vi "Control_1_15.vi"() -> ()   [LabVIEW 2025]
uses:
  <vilib>/addons/zeromq/socket_type.ctl
  <vilib>/DAQmx/write.llb/DAQmx Write (Analog 1D DBL NChan 1Samp).vi
  <vilib>/DAQmx/read.llb/DAQmx Read (Analog DBL 1Chan 1Samp).vi
  <vilib>/DAQmx/read.llb/DAQmx Read (Analog 1D DBL NChan 1Samp).vi
  <vilib>/DAQmx/create/channels.llb/DAQmx Create Channel (AI-Voltage-Basic).vi
  Trimming_Coil_Monitor.vi
  <vilib>/Waveform/DWDTOps.llb/DWDT Digital to Boolean Array.vi
  Trimming_Coil_Command.vi
  <vilib>/DAQmx/miscellaneous.llb/DAQmx Fill In Error Info.vi
  <vilib>/DAQmx/create/channels.llb/DAQmx Create Channel (AO-Voltage-Basic).vi
  Trimming_Coil_Ramps.vi
  <vilib>/addons/zeromq/zmq_socket.lvclass
  <vilib>/addons/zeromq/zmq_context.lvclass
  <vilib>/addons/zeromq/zeromq.lvlib
  <resource>/objmgr/daqmx.rc
panel:
  out "TC6_Ramp":dbl
  out "TC7_Ramp":dbl
  out "x*y":dbl[](array[numeric])
  in  "stop":bool
  out "TC9_Ramp":dbl
  out "TC6_Set_Point":dbl
  out "TC5_Ramp":dbl
  out "TC10_Ramp":dbl
  in  "RF":tag
  in  "Others":tag
  out "error out":errorcluster
  out "double precision float":dbl
  out "Source 1":dbl
  out "Source 2":dbl
  out "Source 3":dbl
  out "Source 4":dbl
  out "Source 5":dbl
  out "Source 6":dbl
  out "Source 7":dbl
  out "Source 8":dbl
  out "Source 9":dbl
  out "Source 10":dbl
  out "Source 11":dbl
  out "Source 12":dbl
  out "Source 13":dbl
  out "Source 14":dbl
  out "value":dbl[](array[numeric])
  out "subarray":dbl[](array[numeric])
  out "Boolean array":bool[](array[boolean])
  out "TC 7":dbl
  out "TC 8":dbl
  in  "Boolean":bool
  out "Array":dbl[](array[numeric])
  out "max value":i16
  out "Array[0]":dbl
  out "Array 2":dbl[](array[numeric])
  in  "TP1":dbl
  in  "TP2":dbl
  in  "RF 2":dbl
  in  "Beam":dbl
  in  "Boolean 2":bool
  in  "Boolean 3":bool
  out "[0]":bool
  out "[1]":bool
  out "[2]":bool
  out "[3]":bool
  out "others":dbl[](array[numeric]) format="%0.2f"
  out "TC1_SP":dbl
  # "Beam I"
  # "ESD KV"
  # "ARC V"
  # "Filament C"
  # "Inside Iron"
  # "Outside Iron"
  # "ARC C"
  # "ESD mA"
  # "TC1"
  # "TC2"
  # "TC4"
  # "TC5"
  # "TC6"
  # "TC7"
  # "TC10"
  # "TC9"
  # "TP2"
  # "TP1"
  # "Filament V"
  # "Centering Beam"
  # "TC 12"
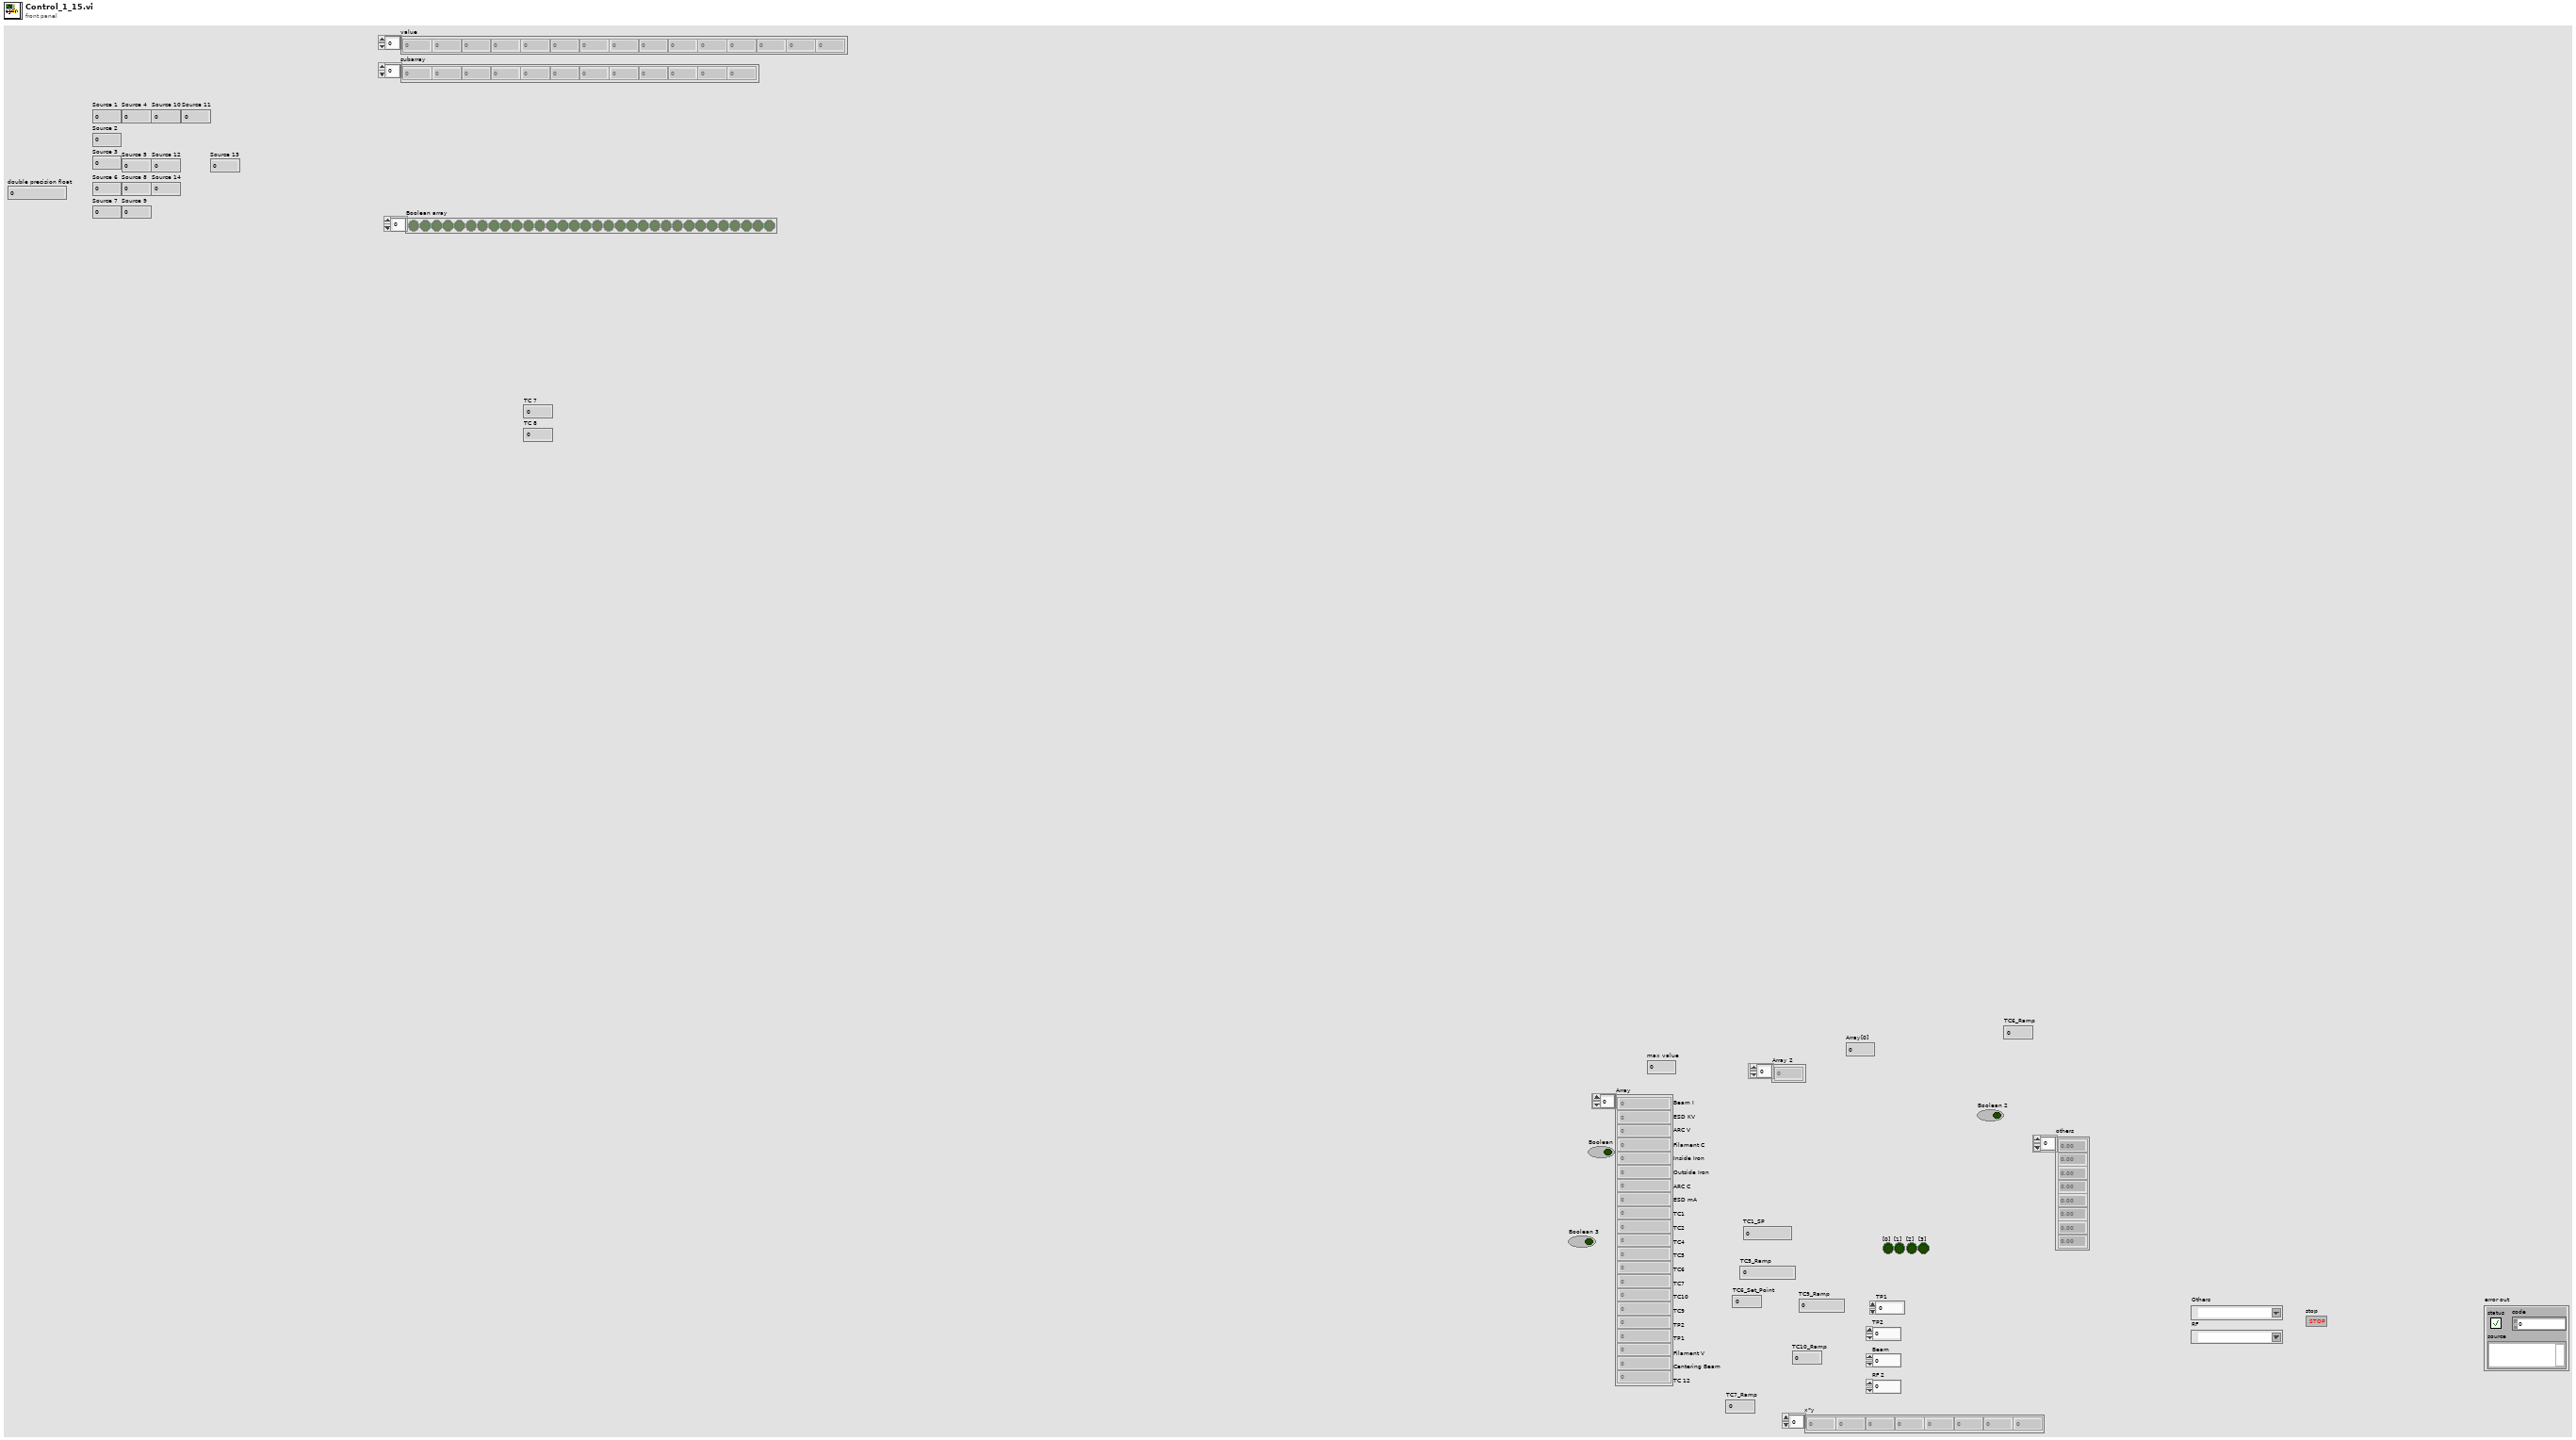
[diagram p1: front panel]
types:
  T1 = typedef "zeromq.lvlib/socket_type.ctl" = enum8{"ZMQ_PAIR", "ZMQ_PUB", "ZMQ_SUB", "ZMQ_REQ", "ZMQ_REP", "ZMQ_DEALER", "ZMQ_ROUTER", "ZMQ_PULL", "ZMQ_PUSH", "ZMQ_XPUB", "ZMQ_XSUB", "ZMQ_STREAM", "ZMQ_SERVER", "ZMQ_CLIENT", "ZMQ_RADIO", "ZMQ_DISH", "ZMQ_GATHER", "ZMQ_SCATTER", "ZMQ_DGRAM"}
  T2 = enum16{"big-endian, network order", "native, host order", "little-endian"}
  T3 = cluster{"[0]":dbl, "[1]":dbl, "[2]":dbl, "[3]":dbl, "[4]":dbl, "[5]":dbl, "[6]":dbl, "[7]":dbl}
  T4 = cluster{"Array[0]":dbl, "Array[1]":dbl, "Array[2]":dbl, "Array[3]":dbl, "Array[4]":dbl, "Array[5]":dbl, "Array[6]":dbl, "Array[7]":dbl}
  T5 = cluster{"[0]":digitalwaveform, "[1]":digitalwaveform, "[2]":digitalwaveform, "[3]":digitalwaveform, "[4]":digitalwaveform, "[5]":digitalwaveform, "[6]":digitalwaveform, "[7]":digitalwaveform, "[8]":digitalwaveform}
  T6 = cluster{"TC1_Readback":dbl, "TC2_Readback":dbl, "TC3_Readback":dbl, "TC4_Readback":dbl, "TC5_Readback":dbl, "TC6_Readback":dbl, "TC7_Readback":dbl, "TC8_Readback":dbl, "TC9_Readback":dbl, "TC10_Readback":dbl, "TC11_Readback":dbl, "TC12_Readback":dbl}
  T7 = cluster{"[0]":bool, "[1]":bool, "[2]":bool, "[3]":bool, "[4]":bool, "[5]":bool, "[6]":bool, "[7]":bool, "[8]":bool}
  T8 = cluster{"TC1_Set_Point":dbl, "TC2_Set_Point":dbl, "TC3_Set_Point":dbl, "TC4_Set_Point":dbl, "TC5_Set_Point":dbl, "TC6_Set_Point":dbl, "TC7_Set_Point":dbl, "TC8_Set_Point":dbl, "TC9_Set_Point":dbl, "TC10_Set_Point":dbl, "TC11_Set_Point":dbl, "TC12_Set_Point":dbl}
  T9 = cluster{"TC1_Ramp":dbl, "TC2_Ramp":dbl, "TC3_Ramp":dbl, "TC4_Ramp":dbl, "TC5_Ramp":dbl, "TC6_Ramp":dbl, "TC7_Ramp":dbl, "TC8_Ramp":dbl, "TC9_Ramp":dbl, "TC10_Ramp":dbl, "TC11_Ramp":dbl, "TC12_Ramp":dbl}
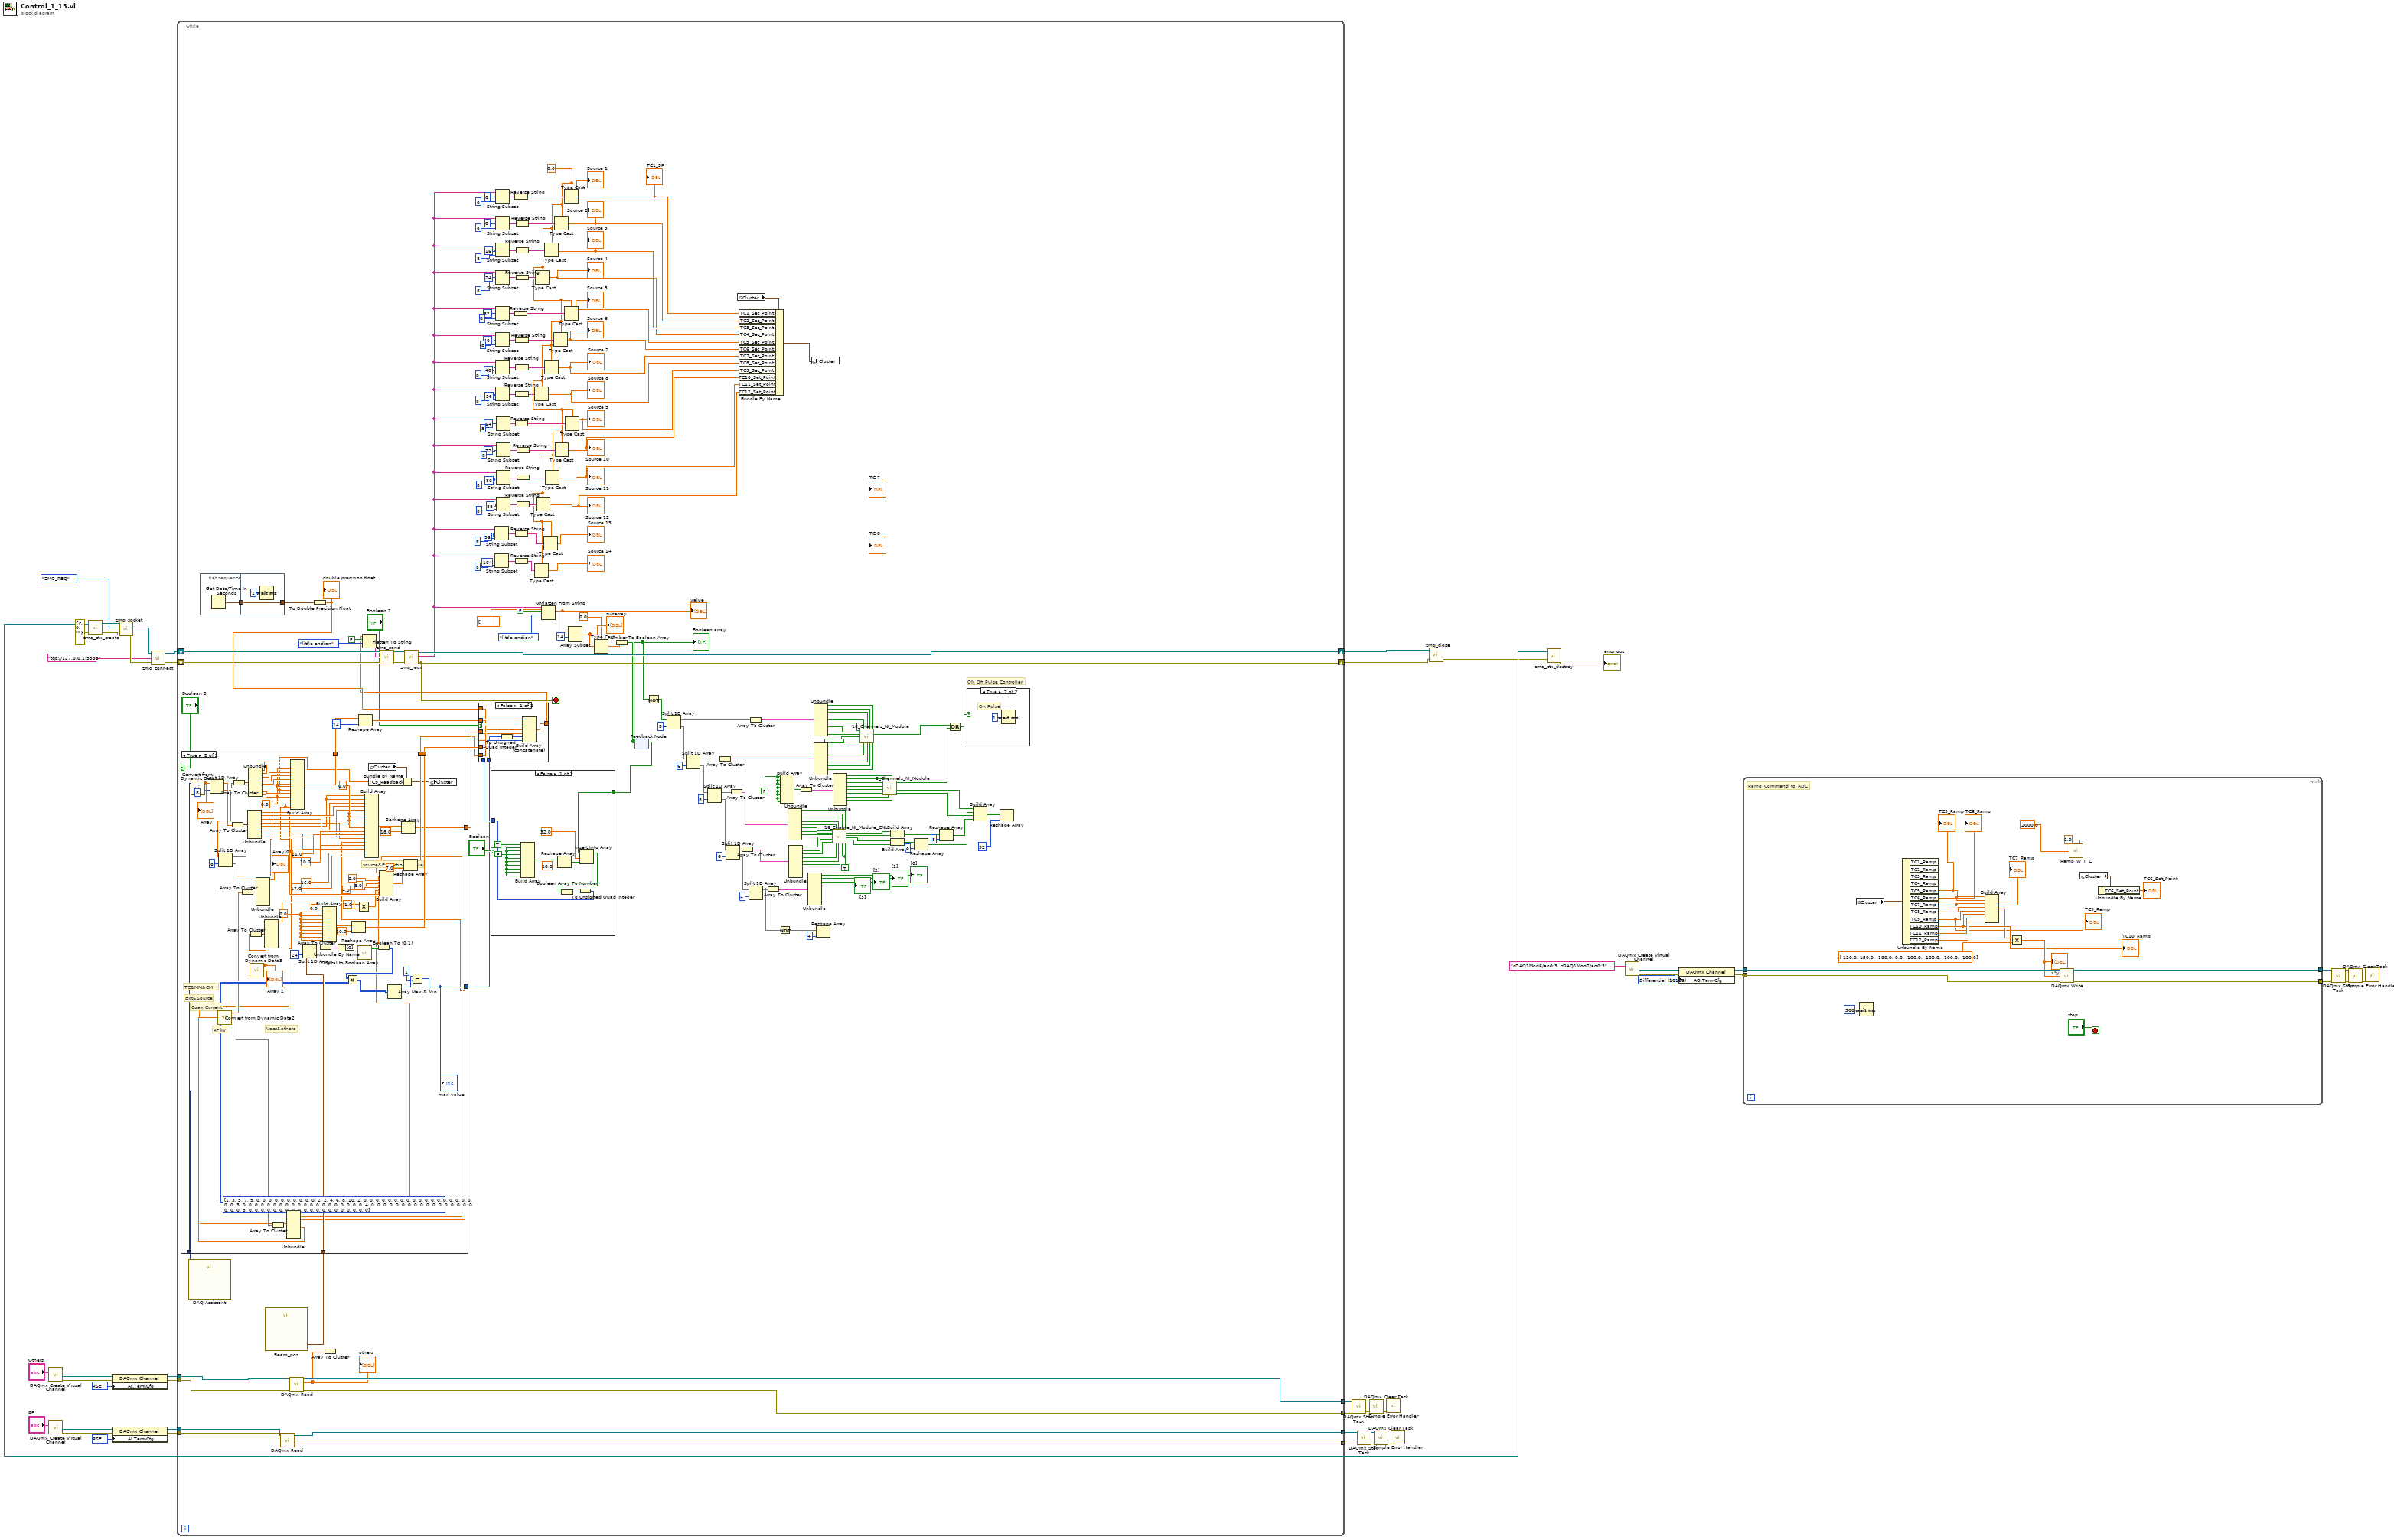
[diagram p0: block diagram]
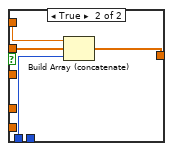
[diagram p2: hidden frame]
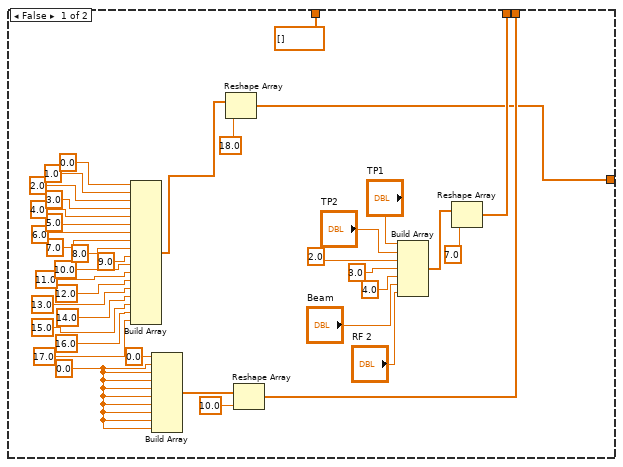
[diagram p3: hidden frame]
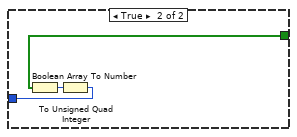
[diagram p4: hidden frame]
diagram:
  w8 = 10106 items=["RSE"=10083, "Differential"=10106, "Pseudodifferential"=12529] ("AO.TermCfg")
  w20 = 10083 items=["RSE"=10083, "Differential"=10106, "Pseudodifferential"=12529] ("AO.TermCfg")
  w31 = 10083 items=["RSE"=10083, "Differential"=10106, "Pseudodifferential"=12529] ("AO.TermCfg")
  n1 = call-poly <vilib>:"DAQmx Create Virtual Channel.vi"("physical channels"="Others") -> ("task out"=w32:refnum<k21>, "error out"=w33:errorcluster)  [unwired: 13 in]
  n2 = call-poly <vilib>:"DAQmx Create Virtual Channel.vi"("physical channels"="RF") -> ("task out"=w21:refnum<k21>, "error out"=w22:errorcluster)  [unwired: 13 in]
  n3 = call <vilib>:"zmq_ctx_create.vi"("error in"=errorcluster {"status"=FALSE, "code"=0, "source"=""}) -> ("error out"=w45:errorcluster, "context out"=w46:refnum<class "zmq_context.lvclass">)  [unwired: 3 in]
  n4 = property class="DAQmx Channel"(reference=w32, error in=w33, "AI.TermCfg"=w31) -> (reference out=w26:refnum<k21>, error out=w25:errorcluster)
  n5 = property class="DAQmx Channel"(reference=w21, error in=w22, "AI.TermCfg"=w20) -> (reference out=w18:refnum<k21>, error out=w17:errorcluster)
  n6 = call <vilib>:"zmq_socket.vi"("error in"=w45, "socket type"=socket_type."ZMQ_REQ", "context in"=w46) -> ("error out"=w43:errorcluster, "socket out"=w44:refnum<class "zmq_socket.lvclass">, "context out"=w38:refnum<class "zmq_context.lvclass">)  [unwired: 2 in]
  n7 = call <vilib>:"zmq_connect.vi"("error in"=w43, "endpoint"="tcp://127.0.0.1:5555", "socket in"=w44) -> ("error out"=w39:errorcluster, "socket out"=w40:refnum<class "zmq_socket.lvclass">)  [unwired: 1 in]
  n8 = while {
    shift-right: [w177] -> w35
    shift-left: w40 -> [w251]
    shift-right: [w176] -> w36
    shift-left: w39 -> [w250]
    tunnel: w26 -> [w77]
    tunnel: w25 -> [w76]
    tunnel: [w75] -> w24
    tunnel: [w74] -> w23
    tunnel: w18 -> [w73]
    tunnel: w17 -> [w72]
    tunnel: [w71] -> w13
    tunnel: [w70] -> w12
    stop <- w176 stop-if-true
    w104 = TRUE
    w107 = FALSE
    w62 = 0.0
    # "ON_Off Pulse Controller"
    n9 = call "DAQ Assistant"() -> ("data"=w64:dynamicdata)  [unwired: 16 in, 3 out]
    n10 = flat-sequence {
      tunnel: [w391] -> w246
      tunnel: [w393] -> w247
      tunnel: w246 -> [w393]
      frame #0 {
        n11 = Get Date/Time In Seconds() -> (seconds since 1Jan1904=w391:timestamp)
      }
      frame #1 {
        n12 = Wait (ms)(milliseconds to wait=u32 1) -> ()  [unwired: 1 out]
      }
    }
    n13 = call "Beam_pos"() -> ("data"=w65:digitalwaveform[])  [unwired: 16 in, 3 out]
    n14 = case shown="True" "Boolean 3" {
      tunnel: [w276 w365] -> w92
      tunnel: [w270 w360] -> w91
      tunnel: [w273 w363] -> w90
      tunnel: w64 -> [_ w357]
      tunnel: [dbl[] [] w358] -> w67
      tunnel: w65 -> [_ w340]
      tunnel: [_ w328] -> w63
      frame False {
        w277 = 0.0 ("element")
        n15 = Build Array(0.0, 1.0, 2.0, 3.0, 4.0, 5.0, 6.0, 7.0, 8.0, 9.0, 10.0, 11.0, 12.0, 13.0, 14.0, 15.0, 16.0, 17.0) -> (w271:dbl[])
        n16 = Build Array(0.0 ("element"), w277, w277, w277, w277, w277, w277, w277, w277, w277) -> (w280:dbl[])
        n17 = Reshape Array(w271, 18.0) -> (w270:dbl[])
        n18 = Reshape Array(w280, 10.0) -> (w276:dbl[])
        n19 = Build Array("TP1", "TP2", 2.0, 3.0, 4.0, "Beam", "RF 2") -> (w274:dbl[])
        n20 = Reshape Array(w274, 7.0) -> (w273:dbl[])
      }
      frame True {
        w307 = 0.0
        w359 = 0.0
        w367 = 0.0 ("element")
        # "RF kV"
        # "Coax Current"
        # "Vacs&others"
        # "Ext&Source"
        # "TC&MM&CM"
        # "source&Extraction&angle"
        n21 = call "Convert from Dynamic Data"("Dynamic Data Type"=w357) -> ("Array"=w348:dbl[])  [unwired: 3 in]
        "Array" <- w348
        n22 = Split 1D Array(array=w348, index=8) -> (first subarray=w311:dbl[], second subarray=w310:dbl[])
        n23 = call "Convert from Dynamic Data2"() -> ("Array"=w330:dbl[])  [unwired: 4 in]
        n24 = Split 1D Array(array=w310, index=8) -> (first subarray=w309:dbl[], second subarray=w318:dbl[])
        n25 = Array To Cluster(array=w311) -> (cluster=w346:T3)
        n26 = Array To Cluster(array=w309) -> (cluster=w349:T3)
        n27 = Array To Cluster(array=w330) -> (cluster=w331:T4)
        n28 = Unbundle(w346) -> ("[0]"=w332:dbl, "[1]"=w345:dbl, "[2]"=w343:dbl, "[3]"=w342:dbl, "[4]"=w312:dbl, "[5]"=w313:dbl, "[6]"=w315:dbl, "[7]"=w344:dbl)
        n29 = Unbundle(w349) -> ("[0]"=w305:dbl, "[1]"=w356:dbl, "[2]"=w355:dbl, "[3]"=w354:dbl, "[4]"=w353:dbl, "[5]"=w352:dbl, "[6]"=w351:dbl, "[7]"=w302:dbl)
        n30 = call "Convert from Dynamic Data3"() -> ("Array"=w323:dbl[])  [unwired: 4 in]
        "Array 2" <- w323
        n31 = Array To Cluster(array=w323) -> (cluster=w324:T4)
        n32 = Unbundle(w331) -> ("Array[0]"=→"Array[0]":dbl)  [unwired: 7 out]
        n33 = Unbundle(w324) -> ("Array[0]"=w322:dbl)  [unwired: 7 out]
        n34 = Array To Cluster(array=w318) -> (cluster=w320:T3)
        n35 = Unbundle(w320) -> ("[0]"=w317:dbl, "[1]"=w316:dbl, "[2]"=w314:dbl, "[3]"=w306:dbl, "[4]"=w308:dbl)  [unwired: 3 out]
        n36 = Build Array(w305, w356, w307, w355, w354, w353, w352, w307, w302, w351, w307, w308, w306, w306) -> (w358:dbl[])
        n37 = Split 1D Array(array=w340, index=24) -> (first subarray=w337:digitalwaveform[])  [unwired: 1 out]
        n38 = Array To Cluster(array=w337) -> (cluster=w339:T5)
        n39 = Build Array(0.0 ("element"), w367, w367, w367, w367, w367, w367, w367, w367, w367) -> (w370:dbl[])
        n40 = Unbundle By Name(w339) -> ("[0]"=w338:digitalwaveform)
        n41 = Reshape Array(w370, 10.0) -> (w365:dbl[])
        n42 = Multiply(x=-1.0, y=w322) -> (x*y=w325:dbl)
        n43 = call-poly <vilib>:"Digital to Boolean Array.vi"("digital waveform"=w338) -> ("boolean array"=w336:bool[][])  [unwired: 9 in, 1 out]
        n44 = Build Array(w312, w312, w313, w345, w344, w359, w359, w359, w359, w359, 10.0, 11.0, w342, w314, w343, w315, 16.0, 17.0) -> (w361:dbl[])
        n45 = global read "Trimming_Coil_Monitor.vi" "Cluster"() -> (w304:T6)
        n46 = Bundle By Name(cluster=w304, "TC9_Readback"=w302) -> (w303:T6)
        n47 = Boolean To (0,1)(Boolean=w336) -> (0, 1=w335:i16[][])
        n48 = Multiply(x=w335, y=i16[][] [[1, 3, 5, 7, 9, 0, 0, 0, 0, 0, 0, 0, 0, 0, 0, 2, 2, 4, 6, 8, 10], [2, 0, 0, 0, 0, 0, 0, 0, 0, 0, 0, 0, 0, 0, 0, 0, 0, 0, 0, 0, 0], [3, 0, 0, 0, 0, 0, 0, 0, 0, 0, 0, 0, 0, 0, 0, 0, 0, 0, 0, 0, 0], [4, 0, 0, 0, 0, 0, 0, 0, 0, 0, 0, 0, 0, 0, 0, 0, 0, 0, 0, 0, 0], [5, 0, 0, 0, 0, 0, 0, 0, 0, 0, 0, 0, 0, 0, 0, 0, 0, 0, 0, 0, 0]]) -> (x*y=w333:i16[][])
        n49 = Build Array(w316, w317, 2.0, 3.0, 4.0, w325, w332) -> (w364:dbl[])
        n50 = Array Max & Min(array=w333) -> (max value=w327:i16)  [unwired: 3 out]
        n51 = Reshape Array(w361, 18.0) -> (w360:dbl[])
        n52 = Reshape Array(w364, 7.0) -> (w363:dbl[])
        n53 = Subtract(x=w327, y=i16 1 ("x")) -> (x-y=w328:i16)
        "max value" <- w328
        n54 = global write "Trimming_Coil_Monitor.vi" "Cluster"(w303) -> ()
      }
    }
    n55 = call-poly <vilib>:"DAQmx Read.vi"("task/channels in"=w73, "error in"=w72) -> ("task out"=w71:refnum<k21>, "error out"=w70:errorcluster)  [unwired: 11 in, 1 out]
    n56 = call-poly <vilib>:"DAQmx Read.vi"("task/channels in"=w77, "error in"=w76) -> ("task out"=w74:refnum<k21>, "data"=w69:dbl[], "error out"=w75:errorcluster)  [unwired: 11 in]
    "others" <- w69
    n57 = To Double Precision Float(number=w247) -> (double precision float=w97:dbl)
    "double precision float" <- w97
    n58 = Array To Cluster(array=w69) -> ()  [unwired: 1 out]
    n59 = Reshape Array(w67, 14 ("dimension size")) -> (w96:dbl[])
    n60 = feedback #1() -> (w100:bool[])  [unwired: 1 in]
    n61 = case shown="False" "Boolean" {
      tunnel: w100 -> [w382 w388]
      tunnel: [w379 w387] -> w98
      frame False {
        w385 = FALSE
        n62 = Build Array(TRUE, w385, w385, w385, w385, w385, w385, w385, w385, w385) -> (w384:bool[])
        n63 = Reshape Array(w384, 10.0) -> (w377:bool[])
        n64 = Insert Into Array(array=w382, index=32.0, new element=w377) -> (w380:bool[])
        n65 = Boolean Array To Number(Boolean array=w380) -> (number=w381:u32)
        n66 = To Unsigned Quad Integer(1:w381) -> (0:w379:u64)
      }
      frame True {
        n67 = Boolean Array To Number(Boolean array=w388) -> (number=w389:u32)
        n68 = To Unsigned Quad Integer(1:w389) -> (0:w387:u64)
      }
    }
    n69 = case shown="False" "Boolean 2" {
      tunnel: w98 -> [w254 w264]
      tunnel: w97 -> [w260 w263]
      tunnel: w96 -> [w259 w262]
      tunnel: [w258 w261] -> w95
      tunnel: w92 -> [w256 _]
      tunnel: w91 -> [w257 _]
      tunnel: w90 -> [w255 _]
      tunnel: w63 -> [w252 _]
      frame False {
        n70 = To Unsigned Quad Integer(1:w252) -> (0:w253:u64)
        n71 = Build Array (concatenate)(w260, w259, w257, w256, w255, w253, w254) -> (w258:dbl[])
      }
      frame True {
        n72 = Build Array (concatenate)(w263, w262, w264) -> (w261:dbl[])
      }
    }
    n73 = Flatten To String(anything=w95, prepend array or string size? (T)=FALSE, byte order (0:big-endian, network order)=T2."little-endian") -> (data string=w175:string)  [unwired: 1 in, 2 out]
    n74 = call <vilib>:"zmq_send.vi"("error in"=w250, "data"=w175, "socket in"=w251) -> ("error out"=w248:errorcluster, "socket out"=w249:refnum<class "zmq_socket.lvclass">)  [unwired: 4 in]
    n75 = call <vilib>:"zmq_recv.vi"("error in"=w248, "socket in"=w249) -> ("error out"=w176:errorcluster, "data"=w174:string, "socket out"=w177:refnum<class "zmq_socket.lvclass">)  [unwired: 3 in, 2 out]
    n76 = String Subset(string=w174, offset (0)=96, length (rest)=8 ("length (rest)")) -> (substring=w191:string)
    n77 = String Subset(string=w174, offset (0)=104, length (rest)=8 ("length (rest)")) -> (substring=w189:string)
    n78 = String Subset(string=w174, offset (0)=32, length (rest)=8 ("length (rest)")) -> (substring=w223:string)
    n79 = String Subset(string=w174, offset (0)=40, length (rest)=8 ("length (rest)")) -> (substring=w221:string)
    n80 = String Subset(string=w174, offset (0)=48, length (rest)=8 ("length (rest)")) -> (substring=w215:string)
    n81 = String Subset(string=w174, offset (0)=56, length (rest)=8 ("length (rest)")) -> (substring=w213:string)
    n82 = String Subset(string=w174, offset (0)=0, length (rest)=8 ("length (rest)")) -> (substring=w239:string)
    n83 = String Subset(string=w174, offset (0)=8, length (rest)=8 ("length (rest)")) -> (substring=w237:string)
    n84 = String Subset(string=w174, offset (0)=16, length (rest)=8 ("length (rest)")) -> (substring=w231:string)
    n85 = String Subset(string=w174, offset (0)=24, length (rest)=8 ("length (rest)")) -> (substring=w229:string)
    n86 = String Subset(string=w174, offset (0)=64, length (rest)=8 ("length (rest)")) -> (substring=w207:string)
    n87 = String Subset(string=w174, offset (0)=72, length (rest)=8 ("length (rest)")) -> (substring=w205:string)
    n88 = String Subset(string=w174, offset (0)=80, length (rest)=8 ("length (rest)")) -> (substring=w199:string)
    n89 = String Subset(string=w174, offset (0)=88, length (rest)=8 ("length (rest)")) -> (substring=w197:string)
    n90 = Reverse String(1:w223) -> (0:w222:string)
    n91 = Reverse String(1:w239) -> (0:w238:string)
    n92 = Reverse String(1:w207) -> (0:w206:string)
    n93 = Reverse String(1:w191) -> (0:w190:string)
    n94 = Reverse String(1:w189) -> (0:w188:string)
    n95 = Reverse String(1:w221) -> (0:w220:string)
    n96 = Reverse String(1:w215) -> (0:w214:string)
    n97 = Reverse String(1:w213) -> (0:w212:string)
    n98 = Reverse String(1:w237) -> (0:w236:string)
    n99 = Reverse String(1:w231) -> (0:w230:string)
    n100 = Reverse String(1:w229) -> (0:w228:string)
    n101 = Reverse String(1:w205) -> (0:w204:string)
    n102 = Reverse String(1:w199) -> (0:w198:string)
    n103 = Reverse String(1:w197) -> (0:w196:string)
    n104 = Type Cast(type=w62, x=w188) -> (*(type *) &x=→"Source 14":dbl)
    n105 = Type Cast(type=w62, x=w212) -> (*(type *) &x=w52:dbl)
    "Source 8" <- w52
    n106 = Type Cast(type=w62, x=w228) -> (*(type *) &x=w56:dbl)
    "Source 4" <- w56
    n107 = Type Cast(type=w62, x=w196) -> (*(type *) &x=w48:dbl)
    "Source 12" <- w48
    n108 = Unflatten From String(type=dbl[] [], binary string=w174, data includes array or string size? (T)=FALSE, byte order (0:big-endian, network order)=T2."little-endian") -> (value=w184:dbl[])  [unwired: 1 in, 2 out]
    "value" <- w184
    n109 = Type Cast(type=w62, x=w190) -> (*(type *) &x=→"Source 13":dbl)
    n110 = Type Cast(type=w62, x=w214) -> (*(type *) &x=w53:dbl)
    "Source 7" <- w53
    n111 = Type Cast(type=w62, x=w230) -> (*(type *) &x=w57:dbl)
    "Source 3" <- w57
    n112 = Type Cast(type=w62, x=w198) -> (*(type *) &x=w49:dbl)
    "Source 11" <- w49
    n113 = Type Cast(type=w62, x=w220) -> (*(type *) &x=w54:dbl)
    "Source 6" <- w54
    n114 = Type Cast(type=w62, x=w236) -> (*(type *) &x=w58:dbl)
    "Source 2" <- w58
    n115 = Type Cast(type=w62, x=w204) -> (*(type *) &x=w50:dbl)
    "Source 10" <- w50
    n116 = Type Cast(type=w62, x=w222) -> (*(type *) &x=w55:dbl)
    "Source 5" <- w55
    n117 = Type Cast(type=w62, x=w238) -> (*(type *) &x=w59:dbl)
    "Source 1" <- w59
    "TC1_SP" <- w59
    n118 = Type Cast(type=w62, x=w206) -> (*(type *) &x=w51:dbl)
    "Source 9" <- w51
    n119 = Array Subset(array=w184, index=14) -> (w182:dbl[])  [unwired: 1 in]
    "subarray" <- w182
    n120 = Type Cast(type=0.0, x=w182) -> (*(type *) &x=w180:dbl)
    n121 = Number To Boolean Array(number=w180) -> (Boolean array=w163:bool[])
    "Boolean array" <- w163
    n122 = feedback-in #1(w163) -> ()
    n123 = Not(x=w163) -> (.not. x?=w162:bool[])
    n124 = Split 1D Array(array=w162, index=8) -> (first subarray=w172:bool[], second subarray=w171:bool[])
    n125 = Split 1D Array(array=w171, index=6) -> (first subarray=w169:bool[], second subarray=w167:bool[])
    n126 = Split 1D Array(array=w167, index=8) -> (first subarray=w166:bool[], second subarray=w164:bool[])
    n127 = Array To Cluster(array=w169) -> (cluster=w142:T7)
    n128 = Split 1D Array(array=w164, index=6) -> (first subarray=w165:bool[], second subarray=w87:bool[])
    n129 = Array To Cluster(array=w166) -> (cluster=w101:T7)
    n130 = global read "Trimming_Coil_Command.vi" "Cluster"() -> (w61:T8)
    n131 = Bundle By Name(cluster=w61, "TC1_Set_Point"=w59, "TC2_Set_Point"=w58, "TC3_Set_Point"=w57, "TC4_Set_Point"=w56, "TC5_Set_Point"=w55, "TC6_Set_Point"=w54, "TC7_Set_Point"=w53, "TC8_Set_Point"=w52, "TC9_Set_Point"=w51, "TC10_Set_Point"=w50, "TC11_Set_Point"=w49, "TC12_Set_Point"=w48) -> (w60:T8)
    n132 = Array To Cluster(array=w165) -> (cluster=w102:T7)
    n133 = Array To Cluster(array=w172) -> (cluster=w145:T7)
    n134 = Split 1D Array(array=w87, index=4) -> (first subarray=w79:bool[])  [unwired: 1 out]
    n135 = Array To Cluster(array=w79) -> (cluster=w86:T7)
    n136 = Not(x=w79) -> (.not. x?=w78:bool[])
    n137 = Build Array(w107, w107, w107, w107, w107, w107, w107, w107) -> (w105:bool[])
    n138 = Unbundle(w101) -> ("[0]"=w131:bool, "[1]"=w130:bool, "[2]"=w129:bool, "[3]"=w128:bool, "[4]"=w127:bool, "[5]"=w126:bool, "[6]"=w125:bool, "[7]"=w124:bool)  [unwired: 1 out]
    n139 = Unbundle(w102) -> ("[0]"=w119:bool, "[1]"=w118:bool, "[2]"=w117:bool, "[3]"=w116:bool, "[4]"=w89:bool, "[5]"=w88:bool)  [unwired: 3 out]
    n140 = Array To Cluster(array=w105) -> (cluster=w106:T7)
    n141 = Unbundle(w86) -> ("[0]"=→"[0]":bool, "[1]"=→"[1]":bool, "[2]"=→"[2]":bool, "[3]"=→"[3]":bool)  [unwired: 5 out]
    n142 = global write "Trimming_Coil_Command.vi" "Cluster"(w60) -> ()
    n143 = Unbundle(w145) -> ("[0]"=w146:bool, "[1]"=w161:bool, "[2]"=w160:bool, "[3]"=w159:bool, "[4]"=w158:bool, "[5]"=w157:bool, "[6]"=w156:bool, "[7]"=w155:bool)  [unwired: 1 out]
    n144 = Unbundle(w142) -> ("[0]"=w154:bool, "[1]"=w153:bool, "[2]"=w152:bool, "[3]"=w151:bool, "[4]"=w150:bool, "[5]"=w149:bool, "[6]"=w148:bool, "[7]"=w147:bool)  [unwired: 1 out]
    n145 = Reshape Array(w78, 4 ("dimension size")) -> ()  [unwired: 1 out]
    n146 = call "16_Enable_NI_Module_CNL.vi"("Enable 6"=w126, "Enable 7"=w125, "Enable 8"=w124, "Enable 9"=w119, "Enable 10"=w118, "Enable 11"=w117, "Enable 5"=w127, "Enable 12"=w116, "Enable 4"=w128, "Enable 13"=w89, "Enable 3"=w129, "Enable 14"=w88, "Enable 2"=w130, "Enable 15"=w104, "Enable 1"=w131, "Enable16"=w104) -> ("9_11_13_15"=w123:bool[], "1_3_5_7"=w122:bool[], "10_12_14_16"=w114:bool[], "2_4_6_8"=w113:bool[])
    n147 = Unbundle(w106) -> ("[0]"=w141:bool, "[1]"=w140:bool, "[2]"=w139:bool, "[3]"=w138:bool, "[4]"=w137:bool, "[5]"=w136:bool, "[6]"=w135:bool, "[7]"=w134:bool)  [unwired: 1 out]
    n148 = call "16_Channels_NI_Module.vi"("Trigger 6"=w157, "Trigger 7"=w156, "Trigger 8"=w155, "Trigger 9"=w154, "Trigger 10"=w153, "Trigger 11"=w152, "Trigger 5"=w158, "Trigger 12"=w151, "Trigger 4"=w159, "Trigger 13"=w150, "Trigger 3"=w160, "Trigger 14"=w149, "Trigger 2"=w161, "Trigger 15"=w148, "Trigger"=w146, "Trigger 16"=w147) -> ("Timing"=w143:bool)  [unwired: 2 in, 1 out]
    n149 = call "8_Channels_NI_Module.vi"("Trigger 8"=w134, "Trigger"=w141, "Trigger 7"=w135, "Trigger 2"=w140, "Trigger 6"=w136, "Trigger 5"=w137, "Trigger 4"=w138, "Trigger 3"=w139) -> ("Off Array"=w132:bool[], "On Array"=w133:bool[], "Timing"=w103:bool)  [unwired: 1 in]
    n150 = Build Array(w123, w122) -> (w120:bool[][])
    n151 = Build Array(w114, w113) -> (w112:bool[][])
    n152 = Reshape Array(w112, 8 ("dimension size")) -> (w108:bool[])
    n153 = Reshape Array(w120, 8 ("dimension size")) -> (w109:bool[])
    n154 = Compound Arithmetic op=OR(w143, w103) -> (w144:bool)
    n155 = case shown="True" w144 {
      frame False {
      }
      frame True {
        # "On Pulse"
        n156 = Wait (ms)(milliseconds to wait=u32 1) -> ()  [unwired: 1 out]
      }
    }
    n157 = Build Array(w133, w108, w132, w109) -> (w111:bool[][])
    n158 = Reshape Array(w111, 32 ("dimension size")) -> ()  [unwired: 1 out]
  }
  n159 = call <vilib>:"DAQmx Stop Task.vi"("task/channels in"=w23, "error in"=w24) -> ("task out"=w29:refnum<k21>, "error out"=w28:errorcluster)  [unwired: 12 in]
  n160 = call <vilib>:"DAQmx Stop Task.vi"("task/channels in"=w13, "error in"=w12) -> ("task out"=w16:refnum<k21>, "error out"=w15:errorcluster)  [unwired: 12 in]
  n161 = call <vilib>:"DAQmx Clear Task.vi"("task in"=w29, "error in"=w28) -> ("error out"=w27:errorcluster)  [unwired: 13 in]
  n162 = call <vilib>:"DAQmx Clear Task.vi"("task in"=w16, "error in"=w15) -> ("error out"=w14:errorcluster)  [unwired: 13 in]
  n163 = call <vilib>:"Simple Error Handler.vi"("error in (no error)"=w27) -> ()  [unwired: 4 in, 5 out]
  n164 = call <vilib>:"Simple Error Handler.vi"("error in (no error)"=w14) -> ()  [unwired: 4 in, 5 out]
  n165 = call <vilib>:"zmq_close.vi"("error in"=w36, "socket"=w35) -> ("error out"=w37:errorcluster)  [unwired: 3 in]
  n166 = call <vilib>:"zmq_ctx_destroy.vi"("error in"=w37, "context in"=w38) -> ("error out"=→"error out":errorcluster)  [unwired: 3 in]
  n167 = call-poly <vilib>:"DAQmx Create Virtual Channel.vi"("physical channels"=tag "cDAQ1Mod6/ao0:3, cDAQ1Mod7/ao0:3") -> ("task out"=w10:refnum<k21>, "error out"=w11:errorcluster)  [unwired: 13 in]
  n168 = property class="DAQmx Channel"(reference=w10, error in=w11, "AO.TermCfg"=w8) -> (reference out=w4:refnum<k21>, error out=w3:errorcluster)
  n169 = while {
    tunnel: w4 -> [w415]
    tunnel: w3 -> [w414]
    tunnel: [w413] -> w2
    tunnel: [w412] -> w1
    stop <- "stop" stop-if-true
    # "Ramp_Command_to_ADC"
    n170 = global read "Trimming_Coil_Ramps.vi" "Cluster"() -> (w405:T9)
    n171 = Wait (ms)(milliseconds to wait=u32 500) -> ()  [unwired: 1 out]
    n172 = Unbundle By Name(w405) -> ("TC5_Ramp"=w396:dbl, "TC6_Ramp"=w410:dbl, "TC7_Ramp"=w409:dbl, "TC8_Ramp"=w408:dbl, "TC9_Ramp"=w398:dbl, "TC10_Ramp"=w400:dbl, "TC11_Ramp"=w407:dbl, "TC12_Ramp"=w406:dbl)  [unwired: 4 out]
    "TC9_Ramp" <- w398
    "TC5_Ramp" <- w396
    "TC10_Ramp" <- w400
    "TC7_Ramp" <- w409
    "TC6_Ramp" <- w410
    n173 = Build Array(w396, w410, w409, w408, w398, w400, w407, w406) -> (w399:dbl[])
    n174 = Multiply(x=w399, y=dbl[] [-120.0, 150.0, -100.0, 0.0, -100.0, -100.0, -100.0, -100.0]) -> (x*y=w404:dbl[])
    "x*y" <- w404
    n175 = call-poly <vilib>:"DAQmx Write.vi"("task/channels in"=w415, "data"=w404, "error in"=w414) -> ("task out"=w413:refnum<k21>, "error out"=w412:errorcluster)  [unwired: 10 in, 1 out]
    n176 = call "Ramp_W_T_C.vi"("Trimming_Coil_Ramp_Error"=1.0, "Trimming_Coil_Ramp_Inc/Dec"=2000.0) -> ()
    n177 = global read "Trimming_Coil_Command.vi" "Cluster"() -> (w403:T8)
    n178 = Unbundle By Name(w403) -> ("TC6_Set_Point"=→"TC6_Set_Point":dbl)
  }
  n179 = call <vilib>:"DAQmx Stop Task.vi"("task/channels in"=w2, "error in"=w1) -> ("task out"=w7:refnum<k21>, "error out"=w6:errorcluster)  [unwired: 12 in]
  n180 = call <vilib>:"DAQmx Clear Task.vi"("task in"=w7, "error in"=w6) -> ("error out"=w5:errorcluster)  [unwired: 13 in]
  n181 = call <vilib>:"Simple Error Handler.vi"("error in (no error)"=w5) -> ()  [unwired: 4 in, 5 out]
